vi "Decode TextString.vi"(7 "Decode from UTF8? (T)":bool=TRUE, 11 "Length-Prefixed Field":u8[](array[numeric]) format="%08x") -> (2 "Text String":string, 3 "Remaining Packets":u8[](array[numeric]) format="%08b", 5 "restricted code":bool)   [LabVIEW 2013, in "MQTT_Control_Packets.lvlib" / "ControlPacket.lvclass"]
uses:
  ControlPacket.lvclass
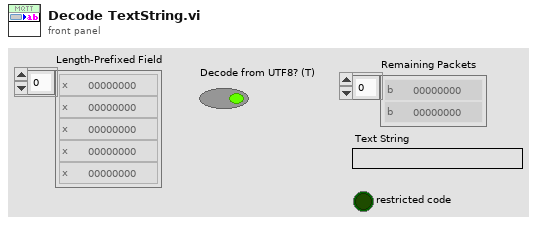
[diagram p1: front panel]
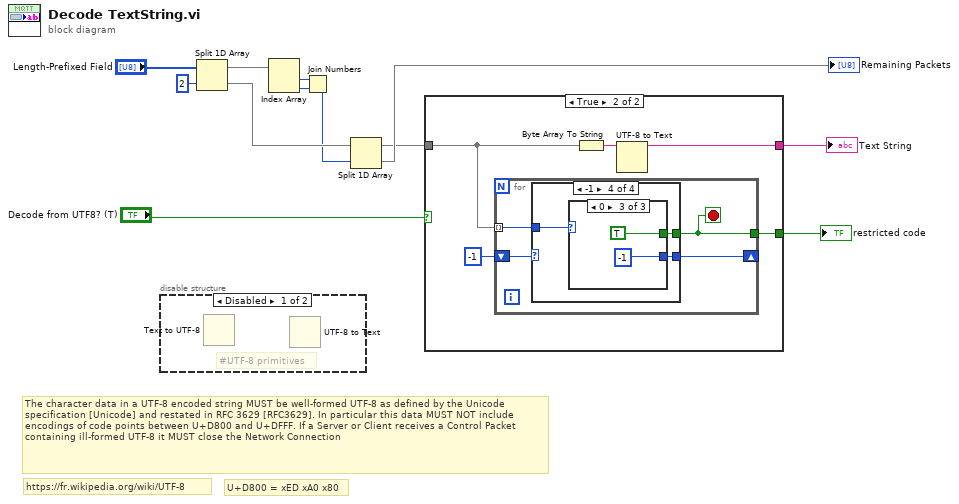
[diagram p0: block diagram]
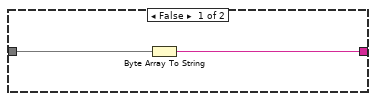
[diagram p2: hidden frame]
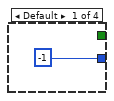
[diagram p3: hidden frame]
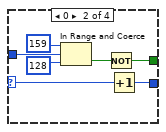
[diagram p4: hidden frame]
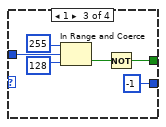
[diagram p5: hidden frame]
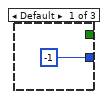
[diagram p6: hidden frame]
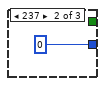
[diagram p7: hidden frame]
diagram:
  # "U+D800 = xED xA0 x80"
  # "https://fr.wikipedia.org/wiki/UTF-8"
  # "The character data in a UTF-8 encoded string MUST be well-formed UTF-8 as defined by the Unicode specification [Unicode] and restated in RFC 3629 [RFC3629]. In particular this data MUST NOT include encodings of code points between U+D800 and U+DFFF. If a Server or Client receives a Control Packet containing ill-formed UTF-8 it MUST close the Network Connection"
  n1 = disable-structure shown="Disabled" {
    frame Disabled {
      # "#UTF-8 primitives"
      n2 = Text to UTF-8() -> ()  [unwired: 2 in, 2 out]
      n3 = UTF-8 to Text() -> ()  [unwired: 2 in, 2 out]
    }
    frame Enabled {
    }
  }
  n4 = Split 1D Array(array="Length-Prefixed Field", index=2) -> (first subarray=w11:u8[], second subarray=w10:u8[])
  n5 = Index Array(array=w11) -> (element #1=w8:u8, element #2=w9:u8)  [unwired: 2 in]
  n6 = Join Numbers(hi=w8, lo=w9) -> ((hi.lo)=w7:u16)
  n7 = Split 1D Array(array=w10, index=w7) -> (first subarray=w4:u8[], second subarray=→"Remaining Packets":u8[])
  n8 = case shown="True" "Decode from UTF8? (T)" {
    tunnel: [w13 w19] -> w6
    tunnel: w4 -> [w14 w17]
    tunnel: [_ w16] -> w3
    frame False {
      n9 = Byte Array To String(unsigned byte array=w14) -> (string=w13:string)
    }
    frame True {
      n10 = for {
        tunnel: w17 -> [w23] mode=indexing
        shift-right: [w22] -> _
        shift-left: -1 -> [w21]
        tunnel: [w20] -> w16
        stop <- w20 stop-if-true
        n11 = case shown="-1" w21 {
          selector: w21 -> [_ w30 _ _]
          tunnel: w23 -> [_ w25 w32 w40]
          tunnel: [-1 w31 -1 w39] -> w22
          tunnel: [_ w26 w34 w38] -> w20
          frame Default {
          }
          frame 0 {
            n12 = In Range and Coerce(upper limit=u8 159 ("Byte"), x=w25, lower limit=u8 128 ("Byte")) -> (In Range?=w27:bool)  [unwired: 1 out]
            n13 = Not(x=w27) -> (.not. x?=w26:bool)
            n14 = Increment(x=w30) -> (x+1=w31:i32)
          }
          frame 1 {
            n15 = In Range and Coerce(upper limit=u8 255 ("Byte"), x=w32, lower limit=u8 128 ("Byte")) -> (In Range?=w35:bool)  [unwired: 1 out]
            n16 = Not(x=w35) -> (.not. x?=w34:bool)
          }
          frame -1 {
            n17 = case shown="0" w40 {
              tunnel: [-1 0 -1] -> w39
              tunnel: [_ _ TRUE] -> w38
              frame Default {
              }
              frame 237 {
              }
              frame 0 {
              }
            }
          }
        }
      }
      n18 = Byte Array To String(unsigned byte array=w17) -> (string=w15:string)
      n19 = UTF-8 to Text(11:w15) -> (3:w19:string)  [unwired: 1 in, 1 out]
    }
  }
  "Text String" <- w6
  "restricted code" <- w3
